vi "VIH Utility - STR - C-Style Escaped String - Parse.vi"(11 "String in":string) -> (3 "String out":string)   [LabVIEW 2014]
doc: "::: VI Helpeks :::\nCopyright (c) 2000-2026 Konstantin Shifershteyn. All rights reserved."
panel:
  # "VI Helpeks\nCopyright (c) 2012-2026 Konstantin Shifershteyn"
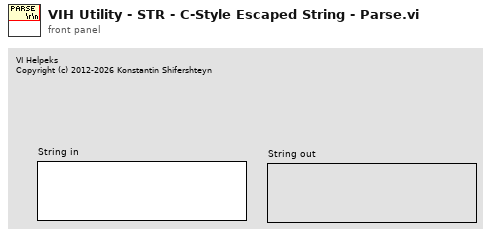
[diagram p1: front panel]
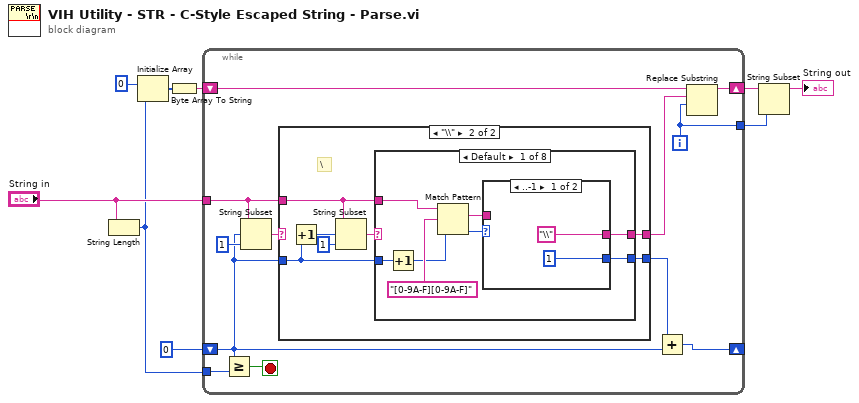
[diagram p0: block diagram]
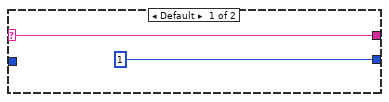
[diagram p2: hidden frame]
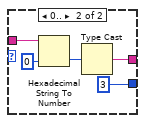
[diagram p3: hidden frame]
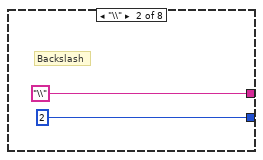
[diagram p4: hidden frame]
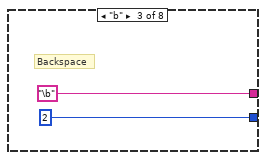
[diagram p5: hidden frame]
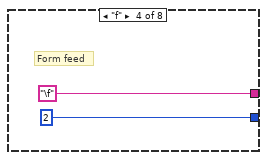
[diagram p6: hidden frame]
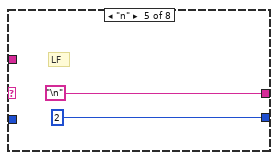
[diagram p7: hidden frame]
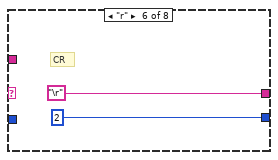
[diagram p8: hidden frame]
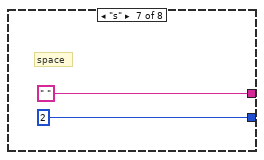
[diagram p9: hidden frame]
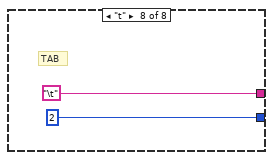
[diagram p10: hidden frame]
diagram:
  n1 = String Length(string="String in") -> (length=w1:i32)
  n2 = Initialize Array(u8 0, w1) -> (w5:u8[])
  n3 = Byte Array To String(unsigned byte array=w5) -> (string=w4:string)
  n4 = while {
    shift-right: [w16] -> _
    shift-left: 0 -> [w12]
    tunnel: "String in" -> [w14]
    shift-right: [w18] -> w3
    shift-left: w4 -> [w19]
    tunnel: [w13] -> w2
    tunnel: w1 -> [w10]
    i -> [w13]
    stop <- w11 stop-if-true
    n5 = Greater Or Equal?(x=w12, y=w10) -> (x >= y?=w11:bool)
    n6 = String Subset(string=w14, offset (0)=w12, length (rest)=1 ("length (rest)")) -> (substring=w20:string)
    n7 = case shown="\"\\\\\"" w20 {
      selector: w20 -> [w23 _]
      tunnel: [w23 w28] -> w17
      tunnel: [1 w27] -> w15
      tunnel: w14 -> [_ w26]
      tunnel: w12 -> [_ w25]
      frame Default {
      }
      frame "\\" {
        # "\\"
        n8 = Increment(x=w25) -> (x+1=w30:i32)
        n9 = String Subset(string=w26, offset (0)=w30, length (rest)=1 ("length (rest)")) -> (substring=w29:string)
        n10 = case shown="Default" w29 {
          tunnel: [w32 "\\" "\b" "\f" "\n" "\r" " " "\t"] -> w28
          tunnel: [w31 2 2 2 2 2 2 2] -> w27
          tunnel: w26 -> [w33 _ _ _ _ _ _ _]
          tunnel: w25 -> [w35 _ _ _ _ _ _ _]
          frame Default {
            n11 = Increment(x=w35) -> (x+1=w34:i32)
            n12 = Match Pattern(string=w33, regular expression="[0-9A-F][0-9A-F]", offset (0)=w34) -> (match substring=w37:string, offset past match=w38:i32)  [unwired: 2 out]
            n13 = case shown="..-1" w38 {
              tunnel: w37 -> [_ w45]
              tunnel: ["\\" w42] -> w32
              tunnel: [1 3] -> w31
              frame ..-1 {
              }
              frame 0.. {
                n14 = Hexadecimal String To Number(string=w45, default (0uL)=u8 0 ("default (0 U32)")) -> (number=w43:u8)  [unwired: 1 in, 1 out]
                n15 = Type Cast(x=w43) -> (*(type *) &x=w42:string)  [unwired: 1 in]
              }
            }
          }
          frame "\\" {
            # "Backslash"
          }
          frame "b" {
            # "Backspace"
          }
          frame "f" {
            # "Form feed"
          }
          frame "n" {
            # "LF"
          }
          frame "r" {
            # "CR"
          }
          frame "s" {
            # "space"
          }
          frame "t" {
            # "TAB"
          }
        }
      }
    }
    n16 = Add(x=w15, y=w12) -> (x+y=w16:i32)
    n17 = Replace Substring(3:w13, 4:w17, 5:w19) -> (1:w18:string)  [unwired: 1 in, 1 out]
  }
  n18 = String Subset(string=w3, length (rest)=w2) -> (substring=→"String out":string)  [unwired: 1 in]
